vi "Read Element of STRANS.vi"(8 "error in (no error)":errorcluster, 10 "index":i32, 11 "Referential in":refnum<class "Referential.lvclass">) -> (0 "error out":errorcluster, 2 "Bit":bool, 3 "Referential out":refnum<class "Referential.lvclass">)   [LabVIEW 2019, in "Referential.lvclass"]
uses:
  Referential.lvclass
  Referential.lvclass/Referential.ctl
  cc7910d5-34f4-4742-907d-8df1f371c4a3.vi/46c8805d-2b02-4896-a6c3-51da333cece9.vi
  <vilib>/Utility/Debug Log/Display.vi
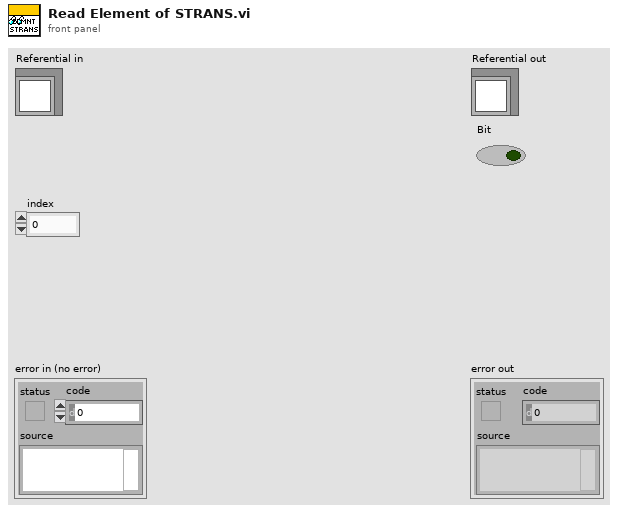
[diagram p1: front panel]
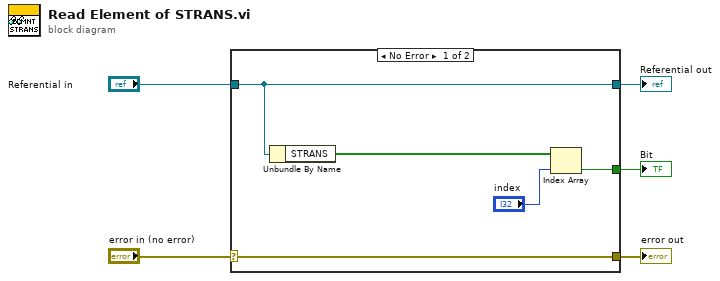
[diagram p0: block diagram]
diagram:
  n1 = case shown="No Error" "error in (no error)" {
    selector: "error in (no error)" -> [w10 w11]
    tunnel: [w10 w11] -> w4
    tunnel: [w9 w12] -> w2
    tunnel: "Referential in" -> [w9 w12]
    tunnel: [w7 _] -> w1
    frame No Error {
      n2 = Unbundle By Name(w9) -> ("STRANS"=w6:bool[])
      n3 = Index Array(array=w6, index="index") -> (element=w7:bool)
    }
    frame Error {
    }
  }
  "error out" <- w4
  "Referential out" <- w2
  "Bit" <- w1
